vi "Read AI physical channels.vi"(8 "error in (no error)":errorcluster, 11 "DAQNavi_AI in":refnum<class "DAQNavi_AI.lvclass">) -> (0 "error out":errorcluster, 2 "physical channels":string="DemoDevice,BID#0/ai0", 3 "DAQNavi_AI out":refnum<class "DAQNavi_AI.lvclass">)   [LabVIEW 2021, in "DAQNavi_AI.lvclass"]
uses:
  DAQNavi_AI.lvclass
  DAQNavi_AI.lvclass/DAQNavi_AI.ctl
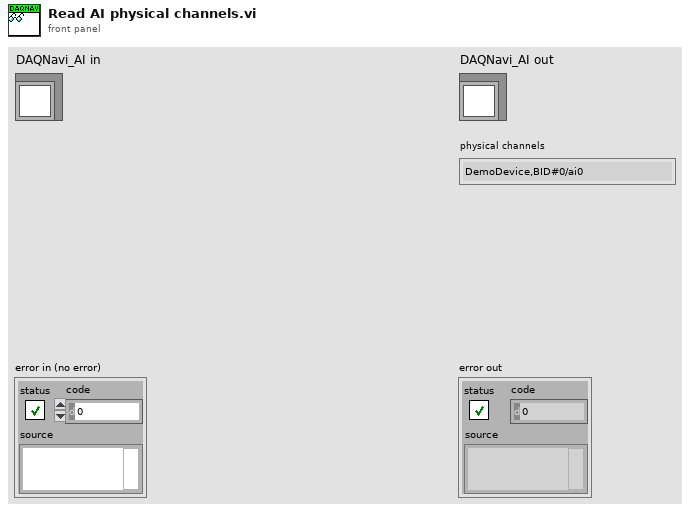
[diagram p1: front panel]
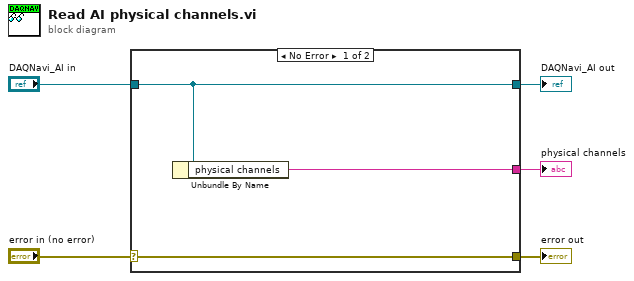
[diagram p0: block diagram]
diagram:
  n1 = case shown="No Error" "error in (no error)" {
    selector: "error in (no error)" -> [w8 w9]
    tunnel: [w8 w9] -> w4
    tunnel: [w7 w10] -> w2
    tunnel: "DAQNavi_AI in" -> [w7 w10]
    tunnel: [w6 _] -> w1
    frame No Error {
      n2 = Unbundle By Name(w7) -> ("physical channels"=w6:string)
    }
    frame Error {
    }
  }
  "error out" <- w4
  "DAQNavi_AI out" <- w2
  "physical channels" <- w1
